vi "VM - Open Context.vi"(6 "close loose contexts (F)":bool, 8 "error in":errorcluster, 10 "context life time":T1, 11 "Creator (top-level VI)":string) -> (0 "error out":errorcluster, 1 "err code":T2 items=["No error", "Invalid variable type", "Variable not found", "Variable already exists", "Invalid context handle", "Input error", "Invalid data format", "No history attached", "History already attached", "Invalid history parameters", "Wrong variable name", "Wrong alias name", "Non-unique alias", "Alias not found", "No alias associated", "Alias already associated", "Wrong context name", "Non-unique context name", "Context name not found", "Invalid parameter", "Generic error", "Memory Full", "Unrecognized LV error", "Unknown error code"], 3 "VC Handle out":T3=-1)   [LabVIEW 2021]
doc: "This VI opens a local variable context. The maximum number of opened contexts is 65535. Refer to the VI help for more details.\n\n<b>VC Handle out</b> indicator returns a handle of the opened context.\n\n::: CalcExpress Toolkit :::\nCopyright (c) 2000-2026 Konstantin Shifershteyn. All rights reserved."
uses:
  cetypes.llb/VarMan Variable Context Handle.ctl
  cetypes.llb/VarMan Error Code.ctl
  cetypes.llb/VarMan Context Life Time.ctl
  cersrc/celveng32.dll
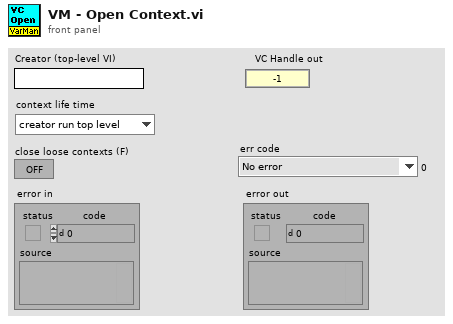
[diagram p1: front panel]
types:
  T1 = typedef "VarMan Context Life Time.ctl" = enum32{"creator run top level", "creator running ", "creator in memory", "untill closed"}
  T2 = typedef "VarMan Error Code.ctl" = u16
  T3 = typedef "VarMan Variable Context Handle.ctl" = i32
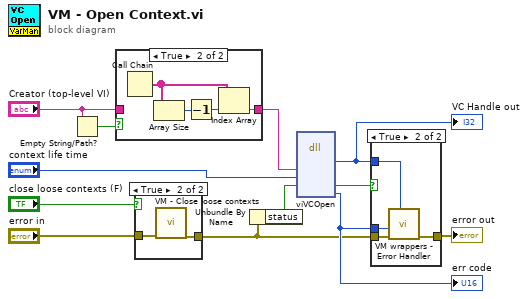
[diagram p0: block diagram]
diagram:
  n1 = Empty String/Path?(string/path="Creator (top-level VI)") -> (empty?=w9:bool)
  n2 = case shown="True" w9 {
    tunnel: [w13 w14] -> w10
    tunnel: "Creator (top-level VI)" -> [w13 _]
    frame False {
    }
    frame True {
      n3 = Call Chain() -> (call chain=w15:string[])
      n4 = Array Size(array=w15) -> (size(s)=w16:i32)
      n5 = Decrement(x=w16) -> (x-1=w17:i32)
      n6 = Index Array(array=w15, index=w17) -> (element=w14:string)
    }
  }
  n7 = case shown="True" "close loose contexts (F)" {
    tunnel: [w18 w20] -> w4
    tunnel: "error in" -> [w18 w19]
    frame False {
    }
    frame True {
      n8 = call "VM - Close loose contexts.vi"("error in"=w19) -> ("error out"=w20:errorcluster)  [unwired: 9 in, 1 out]
    }
  }
  n9 = Unbundle By Name(w4) -> ("status"=w2:bool)
  n10 = dll-call lib="C:/LV Projects/CalcExpress 40 LV2021/vi.lib/addons/CalcExpress/cersrc/celveng*.dll" fn="viVCOpen"("Creator"=w10, "LifeTime"="context life time", "errf"=w2) -> ("VC Handle out"=w11:T3, "errf"=w6:bool, "err code"=w7:T2)  [unwired: 8 in, 2 out]
  "VC Handle out" <- w11
  "err code" <- w7
  n11 = case shown="True" w6 {
    tunnel: [w21 w25] -> w12
    tunnel: w4 -> [w21 w24]
    tunnel: w7 -> [_ w23]
    tunnel: w11 -> [_ w22]
    frame False {
    }
    frame True {
      n12 = call "VM wrappers - Error Handler.vi"("VC Handle"=w22, "error before"=w24, "VarMan error"=w23) -> ("error out"=w25:errorcluster)  [unwired: 7 in, 1 out]
    }
  }
  "error out" <- w12
